vi "BNO055PID.vi"(1 "現偏移角度":dbl=-0.9375, 2 "PID gains":T1={"proportional gain (Kc)"=1.0, "integral time (Ti, min)"=0.0, "derivative time (Td, min)"=0.008} {"derivative time (Td, min)" format="%.3f"; "integral time (Ti, min)" format="%.3f"; "proportional gain (Kc)" format="%.3f"}) -> (0 "ENC":dbl[](array[numeric])=[-0.234375, -0.234375])   [LabVIEW 2019]
uses:
  <vilib>/addons/control/pid/pid.llb/PID (DBL).vi
  <vilib>/addons/control/pid/NI_PID_pid.lvlib
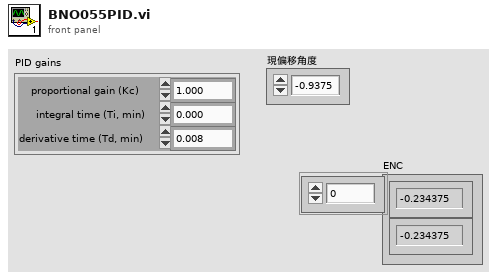
[diagram p1: front panel]
types:
  T1 = cluster{"proportional gain (Kc)":dbl, "integral time (Ti, min)":dbl, "derivative time (Td, min)":dbl}
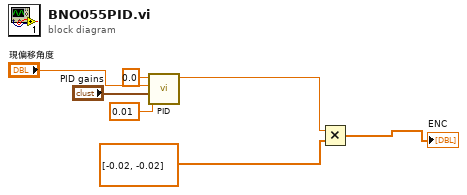
[diagram p0: block diagram]
diagram:
  n1 = call-poly <vilib>:"PID.vi"("dt (s)"=0.01, "PID gains"="PID gains", "process variable"="現偏移角度", "setpoint"=0.0) -> ("output"=w3:dbl)  [unwired: 6 in, 1 out]
  n2 = Multiply(x=w3, y=dbl[] [-0.02, -0.02]) -> (x*y=→"ENC":dbl[])
